vi "I2C An Out M5Stack8ChServo6DOFRobot.vi"() -> ()   [LabVIEW 2020, in "CTI-Scratchpad.lvlib"]
uses:
  CTI-Scratchpad.lvlib
  CTI/Identity.ctl
  CTI/Error Reporting.ctl
  CTI-Peripheral/Analog Output/I2C PWM/M5Stack I2C 8Ch PWM/Private/registers.ctl
  CTI-Peripheral/Analog Output/I2C PWM/M5Stack I2C 8Ch PWM/Private/GPIOOperationModes.ctl
  CTI/I2C Address.ctl
  CTI/GPIO Number.ctl
  CTI/I2C Number.ctl
  3ffc7ce8-1e09-44a0-870a-dca55598b8cb.vi
  734b1e84-ad10-4df0-a8a4-be0d7d03fa5c.vi
  755a3061-6f72-49db-9c25-f728602f264f.vi
  830ba6d0-e88d-4103-9ff4-8f2a25dc46c6.vi
  853c7eef-9088-4e40-91c4-2d7deb58307b.vi
  2fa550b4-2a40-41fb-819f-89677ffc63c5.vi
  ec3d5203-c64e-44e8-9d0a-36cdfa7c2c5f.vi
  CTI/Session/Session.lvclass
  CTI-Peripheral/Analog Output/I2C PWM/M5Stack I2C 8Ch PWM/M5Stack I2C 8Ch Servo.lvclass
  CTI/VisaComms/VisaComms.lvclass
  CTI/CTI.lvlib
panel:
  in  "Rotate to Direction 5":bool
  out "CH5Start":u8
  in  "Rotate to Direction 4":bool
  out "CH4Start":u8
  in  "Move to Direction 3":bool
  out "CH3Start":u8
  in  "Move to Direction 2":bool
  out "CH2Start":u8
  in  "Move to Direction 1":bool
  out "CH1Start":u8
  in  "Middle":bool
  out "CH0Start":u8
  in  "Rotate to Direction 0":bool
  in  "CH7":u8(slide)=90 scale=0.0..180.0
  in  "CH6":u8(slide)=90 scale=0.0..180.0
  in  "CH5":u8(knob) scale=120.0..180.0
  in  "CH4":u8(knob) scale=0.0..180.0
  in  "CH3":u8(knob)
  in  "CH2":u8(knob) scale=0.0..180.0
  in  "CH1":u8(knob) scale=0.0..180.0
  in  "CH0":u8(knob)
  out "loop":i32
  in  "stop":bool
  out "Identity":T1
  in  "Grove Connector":enum16{"I2C0", "I2C1"}(ring)
  out "error out":errorcluster
  in  "Port":refnum<visa-resource-name>="COM4"
  # "https://shop.m5stack.com/products/8-channel-servo-driver-unit-stm32f030?srsltid=AYCX9vJPlmHf0PEe2hkOf9JoORrCSCLFPOOBXTb4mmNWhcA5r_nAQ2T2"
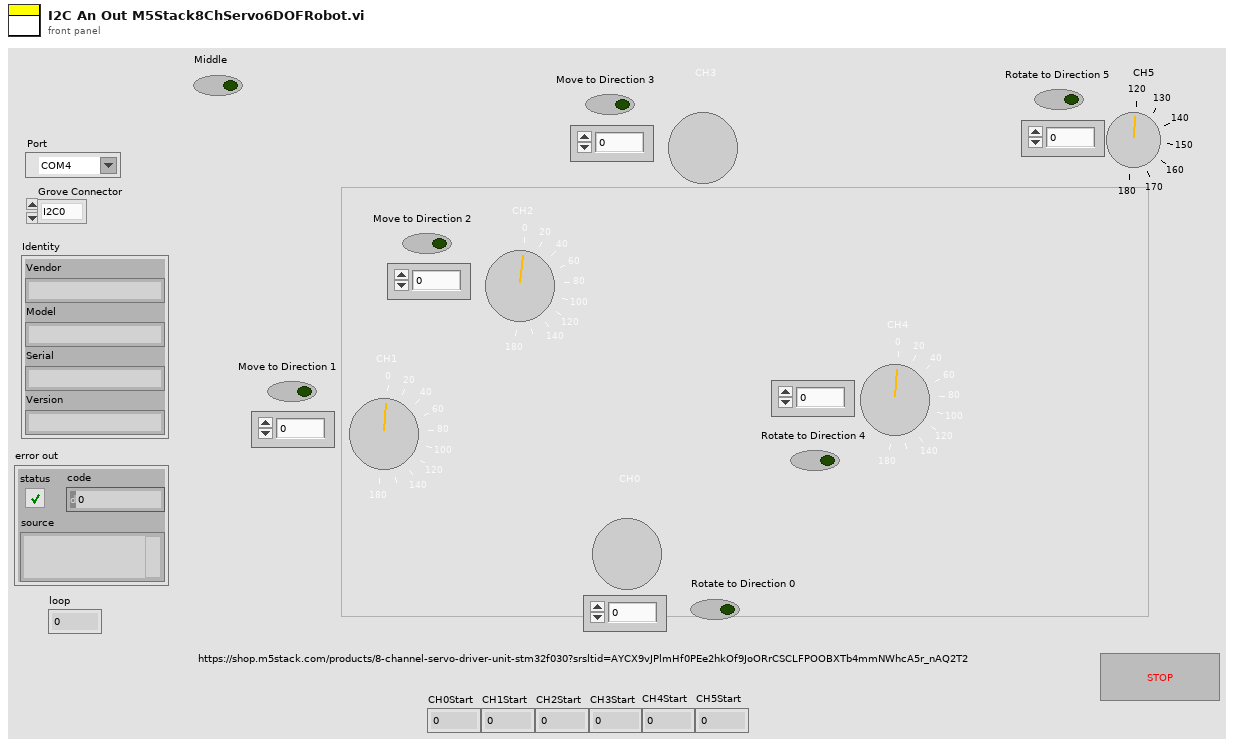
[diagram p1: front panel]
types:
  T1 = typedef "CTI.lvlib/Identity.ctl" = cluster{"Vendor":string, "Model":string, "Serial":string, "Version":string}
  T2 = typedef "CTI.lvlib/I2C Address.ctl" = u8
  T3 = typedef "CTI-Peripheral.lvlib/M5Stack I2C 8Ch Servo.lvclass/GPIOOperationModes.ctl" = u16
  T4 = typedef "CTI-Peripheral.lvlib/M5Stack I2C 8Ch Servo.lvclass/registers.ctl" = u8
  T5 = typedef "CTI.lvlib/Error Reporting.ctl" = enum16{"Minimal", "Moderate", "Full"}
  T6 = typedef "CTI.lvlib/I2C Number.ctl" = i8
  T7 = typedef "CTI.lvlib/GPIO Number.ctl" = i8
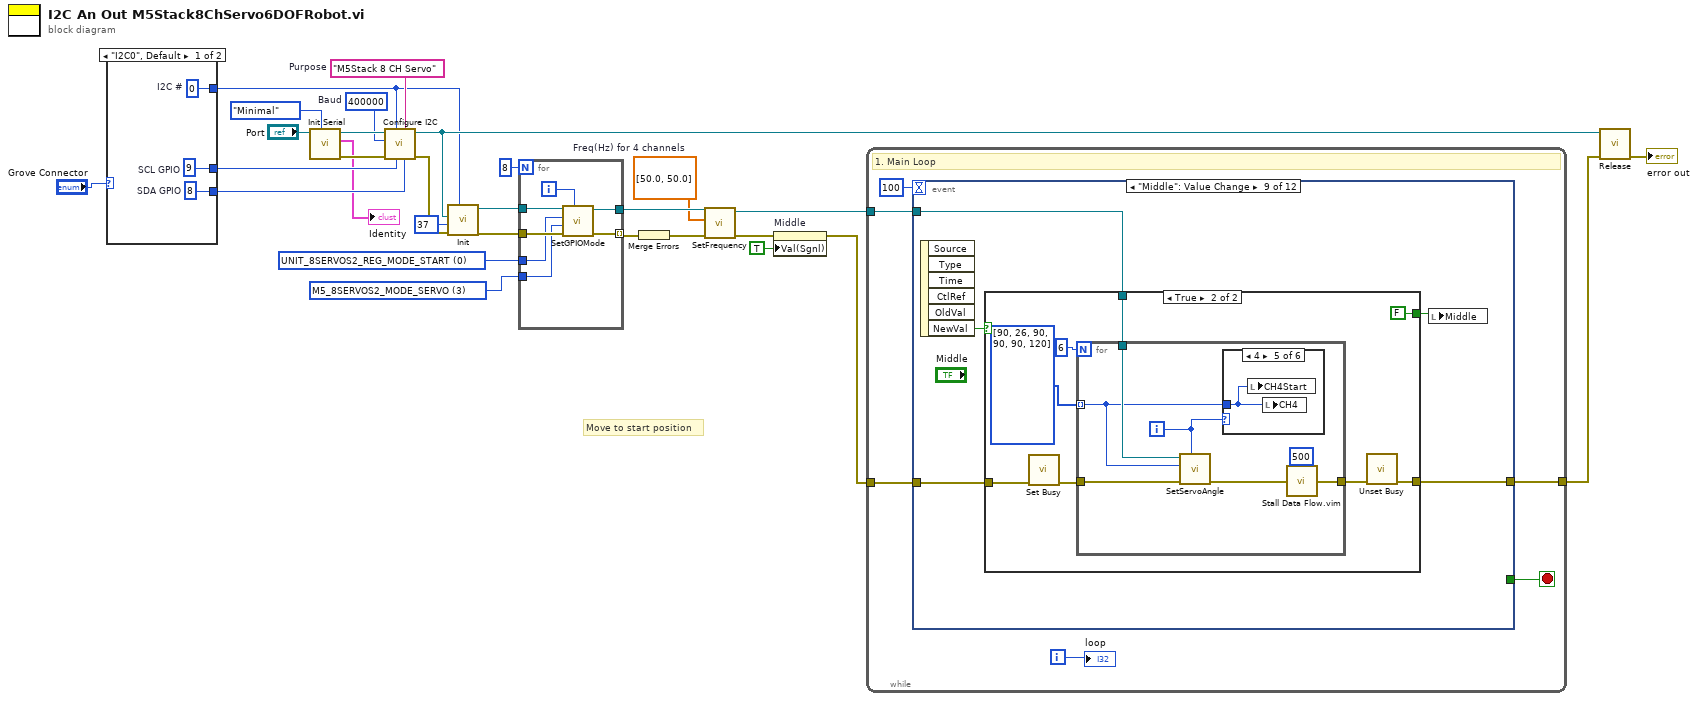
[diagram p0: block diagram]
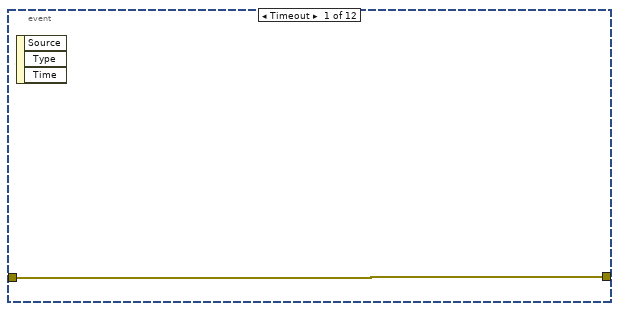
[diagram p2: hidden frame]
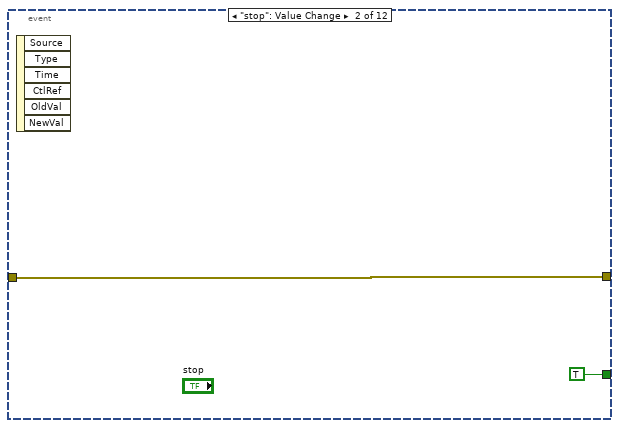
[diagram p3: hidden frame]
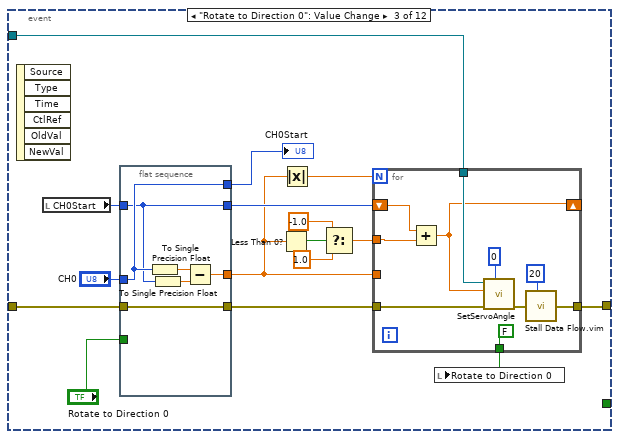
[diagram p4: hidden frame]
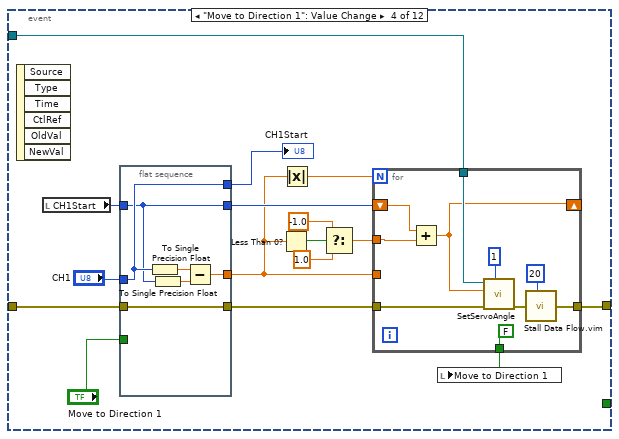
[diagram p5: hidden frame]
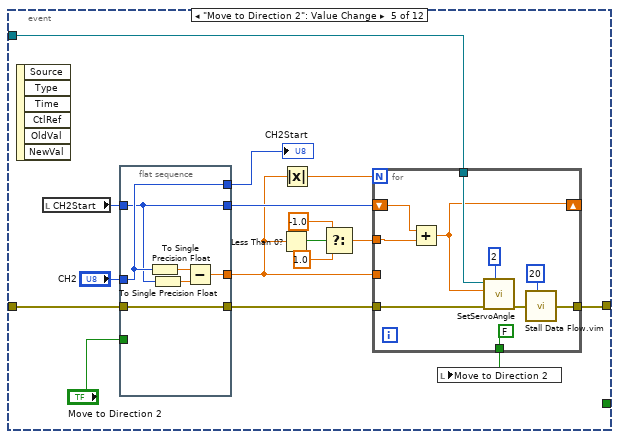
[diagram p6: hidden frame]
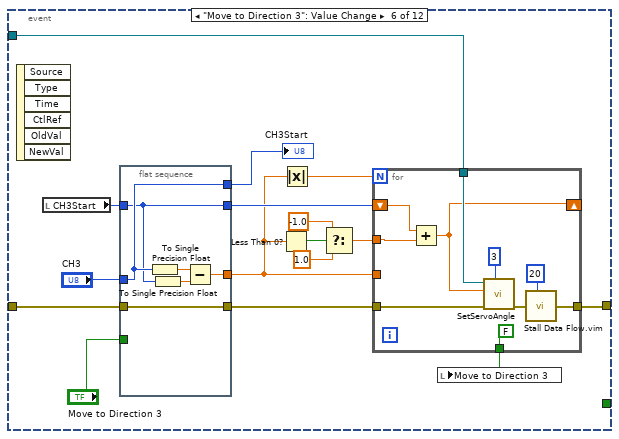
[diagram p7: hidden frame]
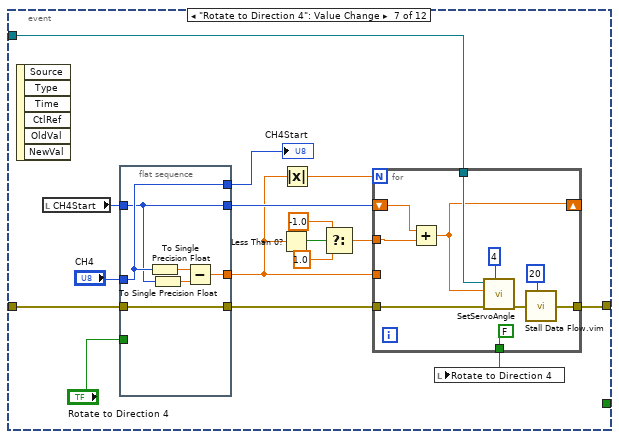
[diagram p8: hidden frame]
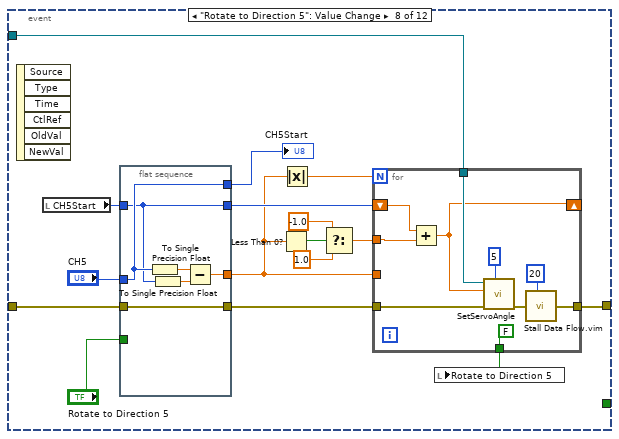
[diagram p9: hidden frame]
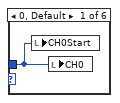
[diagram p11: hidden frame]
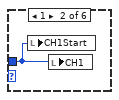
[diagram p12: hidden frame]
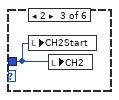
[diagram p13: hidden frame]
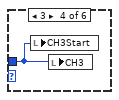
[diagram p14: hidden frame]
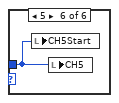
[diagram p15: hidden frame]
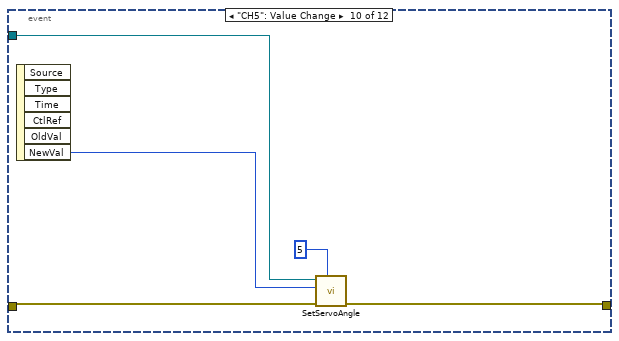
[diagram p16: hidden frame]
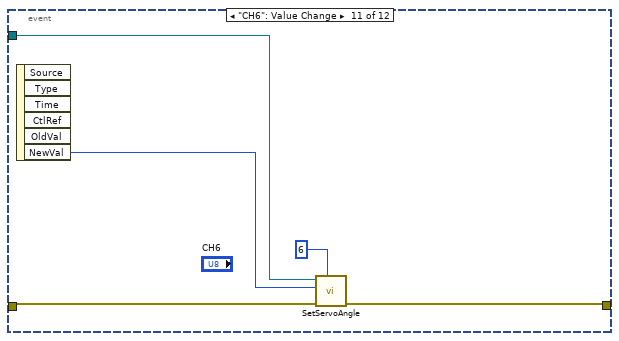
[diagram p17: hidden frame]
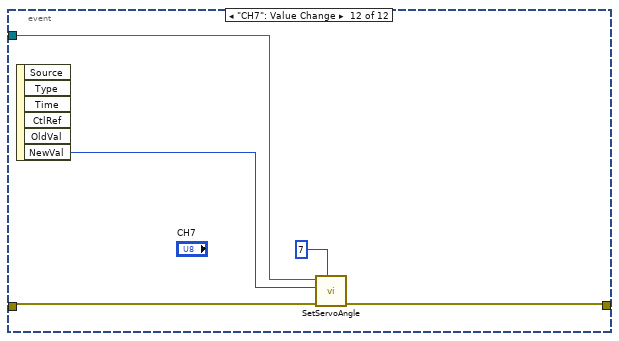
[diagram p18: hidden frame]
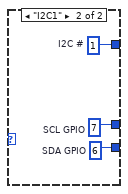
[diagram p19: hidden frame]
diagram:
  w6 = sgl[] [50.0, 50.0]  # Freq(Hz) for 4 channels
  w8 = T3 3 items=["M5_8SERVOS2_MODE_INPUT  ", "M5_8SERVOS2_MODE_OUTPUT ", "M5_8SERVOS2_MODE_ADC    ", "M5_8SERVOS2_MODE_SERVO  ", "M5_8SERVOS2_MODE_RGB    ", "M5_8SERVOS2_MODE_PWM    "] ("Op Mode")
  w9 = T4 0 items=["UNIT_8SERVOS2_REG_MODE_START"=0, "UNIT_8SERVOS2_REG_INPUT_PULL_START"=16, "UNIT_8SERVOS2_REG_INPUT_STATUS_START"=32, "UNIT_8SERVOS2_REG_OUTPUT_STATUS_START"=48, "UNIT_8SERVOS2_REG_ADC_START"=64, "UNIT_8SERVOS2_REG_SERVO_START"=80, "UNIT_8SERVOS2_REG_RGB_CONF_START"=96, "UNIT_8SERVOS2_REG_PWM_DUTY_START"=112, "UNIT_8SERVOS2_REG_RGB_BUFFER_START"=128, "UNIT_8SERVOS2_REG_TIM_FREQ_START"=208, "UNIT_8SERVOS2_REG_UID_START"=224, "UNIT_8SERVOS2_REG_UID_END"=235, "UNIT_8SERVOS2_REG_SYS_ANALOG_START"=240, "UNIT_8SERVOS2_REG_ADDR_OFFSET"=248, "UNIT_8SERVOS2_REG_I2C_ADDR_REFRESH"=252, "UNIT_8SERVOS2_REG_VERSION"=254, "UNIT_8SERVOS2_REG_I2C_ADDR"=255] ("Registers")
  w24 = "M5Stack 8 CH Servo"  # Purpose
  w25 = u32 400000  # Baud
  # "Move to start position"
  n1 = case shown="\"I2C0\", Default" "Grove Connector" {
    tunnel: [w32 w35] -> w22
    tunnel: [w31 w34] -> w21
    tunnel: [w30 w33] -> w15
    frame "I2C0", Default {
      w30 = T6 0  # I2C #
      w31 = T7 8  # SDA GPIO
      w32 = T7 9  # SCL GPIO
    }
    frame "I2C1" {
      w33 = T6 1  # I2C #
      w34 = T7 6  # SDA GPIO
      w35 = T7 7  # SCL GPIO
    }
  }
  n2 = call "Init Serial.vi"("Error Checking (Full)"=Error_Reporting."Minimal", "VISA resource name in"="Port") -> ("error out"=w26:errorcluster, "Identity"=→"Identity":T1, "Session"=w27:refnum<class "Session.lvclass">)  [unwired: 7 in]
  n3 = call "Configure I2C.vi"("SDA GPIO"=w21, "Purpose (\"I2C\")"=w24, "SCL GPIO"=w22, "I2C #"=w15, "error in (no error)"=w26, "Baud"=w25, "Session in"=w27) -> ("error out"=w16:errorcluster, "Session out"=w17:refnum<class "Session.lvclass">)  [unwired: 3 in]
  n4 = call "Init.vi"("I2C #"=w15, "error in (no error)"=w16, "Address"=T2 37, "Session In"=w17) -> ("error out"=w12:errorcluster, "M5Stack8ChPWM Out"=w14:refnum<class "M5Stack I2C 8Ch Servo.lvclass">)  [unwired: 6 in]
  n5 = for {
    N: 8 -> [_]
    tunnel: w14 -> [w42]
    tunnel: w12 -> [w40]
    tunnel: [w39] -> w11 mode=indexing
    tunnel: w9 -> [w38]
    tunnel: w8 -> [w37]
    tunnel: [w36] -> w7
    i -> [w41]
    n6 = call-dynamic "SetGPIOMode.vi"("Channel"=w41, "error in (no error)"=w40, "Op Mode"=w37, "Registers"=w38, "M5Stack I2C 8Ch Servo in"=w42) -> ("error out"=w39:errorcluster, "M5Stack I2C 8Ch Servo out"=w36:refnum<class "M5Stack I2C 8Ch Servo.lvclass">)  [unwired: 5 in]
  }
  n7 = Merge Errors(w11) -> (w10:errorcluster)
  n8 = call-dynamic "SetFrequency.vi"("error in (no error)"=w10, "Freq"=w6, "M5Stack I2C 8Ch Servo in"=w7) -> ("error out"=w3:errorcluster, "M5Stack I2C 8Ch Servo out"=w4:refnum<class "M5Stack I2C 8Ch Servo.lvclass">)  [unwired: 7 in]
  n9 = property on="Middle" class="Bool (strict)"(error in=w3, "Val(Sgnl)"=TRUE ("Value (Signaling)")) -> (error out=w2:errorcluster)  [unwired: 1 in, 1 out]
  n10 = while {
    tunnel: w2 -> [w47]
    tunnel: w4 -> [w48]
    tunnel: [w45] -> w19
    i -> [w46]
    stop <- w44 stop-if-true
    # "1. Main Loop"
    n11 = event shown="[8] \"Middle\": Value Change" {
      selector: _ -> [_ _ _ _ _ _ _ _ _ _ _ _]
      dyn-events: _ -> [_ _ _ _ _ _ _ _ _ _ _ _]
      timeout: 100 -> [_ _ _ _ _ _ _ _ _ _ _ _]
      tunnel: w48 -> [_ _ w67 w99 w131 w163 w195 w227 w247 w273 w278 w283]
      tunnel: w47 -> [w49 w50 w65 w97 w129 w161 w193 w225 w248 w275 w280 w285]
      tunnel: [w49 w50 w66 w98 w130 w162 w194 w226 w246 w274 w279 w284] -> w45
      tunnel: [_ TRUE _ _ _ _ _ _ _ _ _ _] -> w44
      event Timeout {
        n12 = event-data() -> ()  [unwired: 1 in, 3 out]
      }
      event "stop": Value Change {
        n13 = event-data() -> ()  [unwired: 1 in, 6 out]
      }
      event "Rotate to Direction 0": Value Change {
        n14 = event-data() -> ()  [unwired: 1 in, 6 out]
        n15 = local read "CH0Start"() -> (w63:u8)
        n16 = flat-sequence {
          tunnel: w65 -> [w73]
          tunnel: "CH0" -> [w72]
          tunnel: w63 -> [w71]
          tunnel: [w73] -> w62
          tunnel: [w72] -> w61
          tunnel: [w71] -> w60
          tunnel: [w70] -> w58
          tunnel: "Rotate to Direction 0" -> [_]
          frame #0 {
            n17 = To Single Precision Float(number=w72) -> (single precision float=w68:sgl)
            n18 = To Single Precision Float(number=w71) -> (single precision float=w69:sgl)
            n19 = Subtract(x=w68, y=w69) -> (x-y=w70:sgl)
          }
        }
        n20 = Less Than 0?(x=w58) -> (x < 0?=w57:bool)
        n21 = Absolute Value(x=w58) -> (abs(x)=w59:sgl)
        n22 = Select(t=-1.0, s=w57, f=1.0) -> (s? t:f=w54:dbl)
        n23 = for {
          N: w59 -> [_]
          tunnel: w67 -> [w82]
          tunnel: w62 -> [w83]
          tunnel: [w79] -> w66
          tunnel: w58 -> [_]
          shift-right: [w75] -> _
          shift-left: w60 -> [w76]
          tunnel: w54 -> [w77]
          tunnel: [FALSE] -> w52
          n24 = Add(x=w76, y=w77) -> (x+y=w75:dbl)
          n25 = call-dynamic "SetServoAngle.vi"("Channel"=u8 0, "error in (no error)"=w83, "Angle"=w75, "M5Stack I2C 8Ch Servo in"=w82) -> ("error out"=w80:errorcluster)  [unwired: 6 in, 1 out]
          n26 = call "Stall Data Flow.vim"("value in"=w80, "milliseconds to wait"=u32 20) -> ("value out"=w79:errorcluster)  [unwired: 1 out]
        }
        n27 = local write "Rotate to Direction 0"(w52) -> ()
        "CH0Start" <- w61
      }
      event "Move to Direction 1": Value Change {
        n28 = event-data() -> ()  [unwired: 1 in, 6 out]
        n29 = local read "CH1Start"() -> (w96:u8)
        n30 = flat-sequence {
          tunnel: w97 -> [w105]
          tunnel: "CH1" -> [w104]
          tunnel: w96 -> [w103]
          tunnel: [w105] -> w95
          tunnel: [w104] -> w94
          tunnel: [w103] -> w93
          tunnel: [w102] -> w91
          tunnel: "Move to Direction 1" -> [_]
          frame #0 {
            n31 = To Single Precision Float(number=w104) -> (single precision float=w100:sgl)
            n32 = To Single Precision Float(number=w103) -> (single precision float=w101:sgl)
            n33 = Subtract(x=w100, y=w101) -> (x-y=w102:sgl)
          }
        }
        n34 = Less Than 0?(x=w91) -> (x < 0?=w90:bool)
        n35 = Absolute Value(x=w91) -> (abs(x)=w92:sgl)
        n36 = Select(t=-1.0, s=w90, f=1.0) -> (s? t:f=w87:dbl)
        n37 = for {
          N: w92 -> [_]
          tunnel: w99 -> [w114]
          tunnel: w95 -> [w115]
          tunnel: [w111] -> w98
          tunnel: w91 -> [_]
          shift-right: [w107] -> _
          shift-left: w93 -> [w108]
          tunnel: w87 -> [w109]
          tunnel: [FALSE] -> w85
          n38 = Add(x=w108, y=w109) -> (x+y=w107:dbl)
          n39 = call-dynamic "SetServoAngle.vi"("Channel"=u8 1, "error in (no error)"=w115, "Angle"=w107, "M5Stack I2C 8Ch Servo in"=w114) -> ("error out"=w112:errorcluster)  [unwired: 6 in, 1 out]
          n40 = call "Stall Data Flow.vim"("value in"=w112, "milliseconds to wait"=u32 20) -> ("value out"=w111:errorcluster)  [unwired: 1 out]
        }
        n41 = local write "Move to Direction 1"(w85) -> ()
        "CH1Start" <- w94
      }
      event "Move to Direction 2": Value Change {
        n42 = event-data() -> ()  [unwired: 1 in, 6 out]
        n43 = local read "CH2Start"() -> (w128:u8)
        n44 = flat-sequence {
          tunnel: w129 -> [w137]
          tunnel: "CH2" -> [w136]
          tunnel: w128 -> [w135]
          tunnel: [w137] -> w127
          tunnel: [w136] -> w126
          tunnel: [w135] -> w125
          tunnel: [w134] -> w123
          tunnel: "Move to Direction 2" -> [_]
          frame #0 {
            n45 = To Single Precision Float(number=w136) -> (single precision float=w132:sgl)
            n46 = To Single Precision Float(number=w135) -> (single precision float=w133:sgl)
            n47 = Subtract(x=w132, y=w133) -> (x-y=w134:sgl)
          }
        }
        n48 = Less Than 0?(x=w123) -> (x < 0?=w122:bool)
        n49 = Absolute Value(x=w123) -> (abs(x)=w124:sgl)
        n50 = Select(t=-1.0, s=w122, f=1.0) -> (s? t:f=w119:dbl)
        n51 = for {
          N: w124 -> [_]
          tunnel: w131 -> [w146]
          tunnel: w127 -> [w147]
          tunnel: [w143] -> w130
          tunnel: w123 -> [_]
          shift-right: [w139] -> _
          shift-left: w125 -> [w140]
          tunnel: w119 -> [w141]
          tunnel: [FALSE] -> w117
          n52 = Add(x=w140, y=w141) -> (x+y=w139:dbl)
          n53 = call-dynamic "SetServoAngle.vi"("Channel"=u8 2, "error in (no error)"=w147, "Angle"=w139, "M5Stack I2C 8Ch Servo in"=w146) -> ("error out"=w144:errorcluster)  [unwired: 6 in, 1 out]
          n54 = call "Stall Data Flow.vim"("value in"=w144, "milliseconds to wait"=u32 20) -> ("value out"=w143:errorcluster)  [unwired: 1 out]
        }
        n55 = local write "Move to Direction 2"(w117) -> ()
        "CH2Start" <- w126
      }
      event "Move to Direction 3": Value Change {
        n56 = event-data() -> ()  [unwired: 1 in, 6 out]
        n57 = local read "CH3Start"() -> (w160:u8)
        n58 = flat-sequence {
          tunnel: w161 -> [w169]
          tunnel: "CH3" -> [w168]
          tunnel: w160 -> [w167]
          tunnel: [w169] -> w159
          tunnel: [w168] -> w158
          tunnel: [w167] -> w157
          tunnel: [w166] -> w155
          tunnel: "Move to Direction 3" -> [_]
          frame #0 {
            n59 = To Single Precision Float(number=w168) -> (single precision float=w164:sgl)
            n60 = To Single Precision Float(number=w167) -> (single precision float=w165:sgl)
            n61 = Subtract(x=w164, y=w165) -> (x-y=w166:sgl)
          }
        }
        n62 = Less Than 0?(x=w155) -> (x < 0?=w154:bool)
        n63 = Absolute Value(x=w155) -> (abs(x)=w156:sgl)
        n64 = Select(t=-1.0, s=w154, f=1.0) -> (s? t:f=w151:dbl)
        n65 = for {
          N: w156 -> [_]
          tunnel: w163 -> [w178]
          tunnel: w159 -> [w179]
          tunnel: [w175] -> w162
          tunnel: w155 -> [_]
          shift-right: [w171] -> _
          shift-left: w157 -> [w172]
          tunnel: w151 -> [w173]
          tunnel: [FALSE] -> w149
          n66 = Add(x=w172, y=w173) -> (x+y=w171:dbl)
          n67 = call-dynamic "SetServoAngle.vi"("Channel"=u8 3, "error in (no error)"=w179, "Angle"=w171, "M5Stack I2C 8Ch Servo in"=w178) -> ("error out"=w176:errorcluster)  [unwired: 6 in, 1 out]
          n68 = call "Stall Data Flow.vim"("value in"=w176, "milliseconds to wait"=u32 20) -> ("value out"=w175:errorcluster)  [unwired: 1 out]
        }
        n69 = local write "Move to Direction 3"(w149) -> ()
        "CH3Start" <- w158
      }
      event "Rotate to Direction 4": Value Change {
        n70 = event-data() -> ()  [unwired: 1 in, 6 out]
        n71 = local read "CH4Start"() -> (w192:u8)
        n72 = flat-sequence {
          tunnel: w193 -> [w201]
          tunnel: "CH4" -> [w200]
          tunnel: w192 -> [w199]
          tunnel: [w201] -> w191
          tunnel: [w200] -> w190
          tunnel: [w199] -> w189
          tunnel: [w198] -> w187
          tunnel: "Rotate to Direction 4" -> [_]
          frame #0 {
            n73 = To Single Precision Float(number=w200) -> (single precision float=w196:sgl)
            n74 = To Single Precision Float(number=w199) -> (single precision float=w197:sgl)
            n75 = Subtract(x=w196, y=w197) -> (x-y=w198:sgl)
          }
        }
        n76 = Less Than 0?(x=w187) -> (x < 0?=w186:bool)
        n77 = Absolute Value(x=w187) -> (abs(x)=w188:sgl)
        n78 = Select(t=-1.0, s=w186, f=1.0) -> (s? t:f=w183:dbl)
        n79 = for {
          N: w188 -> [_]
          tunnel: w195 -> [w210]
          tunnel: w191 -> [w211]
          tunnel: [w207] -> w194
          tunnel: w187 -> [_]
          shift-right: [w203] -> _
          shift-left: w189 -> [w204]
          tunnel: w183 -> [w205]
          tunnel: [FALSE] -> w181
          n80 = Add(x=w204, y=w205) -> (x+y=w203:dbl)
          n81 = call-dynamic "SetServoAngle.vi"("Channel"=u8 4, "error in (no error)"=w211, "Angle"=w203, "M5Stack I2C 8Ch Servo in"=w210) -> ("error out"=w208:errorcluster)  [unwired: 6 in, 1 out]
          n82 = call "Stall Data Flow.vim"("value in"=w208, "milliseconds to wait"=u32 20) -> ("value out"=w207:errorcluster)  [unwired: 1 out]
        }
        n83 = local write "Rotate to Direction 4"(w181) -> ()
        "CH4Start" <- w190
      }
      event "Rotate to Direction 5": Value Change {
        n84 = event-data() -> ()  [unwired: 1 in, 6 out]
        n85 = local read "CH5Start"() -> (w224:u8)
        n86 = flat-sequence {
          tunnel: w225 -> [w233]
          tunnel: "CH5" -> [w232]
          tunnel: w224 -> [w231]
          tunnel: [w233] -> w223
          tunnel: [w232] -> w222
          tunnel: [w231] -> w221
          tunnel: [w230] -> w219
          tunnel: "Rotate to Direction 5" -> [_]
          frame #0 {
            n87 = To Single Precision Float(number=w232) -> (single precision float=w228:sgl)
            n88 = To Single Precision Float(number=w231) -> (single precision float=w229:sgl)
            n89 = Subtract(x=w228, y=w229) -> (x-y=w230:sgl)
          }
        }
        n90 = Less Than 0?(x=w219) -> (x < 0?=w218:bool)
        n91 = Absolute Value(x=w219) -> (abs(x)=w220:sgl)
        n92 = Select(t=-1.0, s=w218, f=1.0) -> (s? t:f=w215:dbl)
        n93 = for {
          N: w220 -> [_]
          tunnel: w227 -> [w242]
          tunnel: w223 -> [w243]
          tunnel: [w239] -> w226
          tunnel: w219 -> [_]
          shift-right: [w235] -> _
          shift-left: w221 -> [w236]
          tunnel: w215 -> [w237]
          tunnel: [FALSE] -> w213
          n94 = Add(x=w236, y=w237) -> (x+y=w235:dbl)
          n95 = call-dynamic "SetServoAngle.vi"("Channel"=u8 5, "error in (no error)"=w243, "Angle"=w235, "M5Stack I2C 8Ch Servo in"=w242) -> ("error out"=w240:errorcluster)  [unwired: 6 in, 1 out]
          n96 = call "Stall Data Flow.vim"("value in"=w240, "milliseconds to wait"=u32 20) -> ("value out"=w239:errorcluster)  [unwired: 1 out]
        }
        n97 = local write "Rotate to Direction 5"(w213) -> ()
        "CH5Start" <- w222
      }
      event "Middle": Value Change {
        n98 = event-data() -> ("NewVal"=w245:bool)  [unwired: 1 in, 5 out]
        n99 = case shown="True" w245 {
          tunnel: w248 -> [w249 w257]
          tunnel: w247 -> [_ w255]
          tunnel: [w249 w252] -> w246
          tunnel: [_ FALSE] -> w244
          frame False {
          }
          frame True {
            n100 = call <vilib>:"Set Busy.vi"("error in (no error)"=w257) -> ("error out"=w253:errorcluster)  [unwired: 9 in, 1 out]
            n101 = for {
              N: 6 -> [_]
              tunnel: w255 -> [w262]
              tunnel: w253 -> [w264]
              tunnel: [w261] -> w256
              tunnel: u8[] [90, 26, 90, 90, 90, 120] -> [w258] mode=indexing
              i -> [w259]
              n102 = call-dynamic "SetServoAngle.vi"("Channel"=w259, "error in (no error)"=w264, "Angle"=w258, "M5Stack I2C 8Ch Servo in"=w262) -> ("error out"=w263:errorcluster)  [unwired: 6 in, 1 out]
              n103 = case shown="4" w259 {
                tunnel: w258 -> [w265 w266 w267 w268 w269 w270]
                frame 0, Default {
                  n104 = local write "CH0Start"(w265) -> ()
                  n105 = local write "CH0"(w265) -> ()
                }
                frame 1 {
                  n106 = local write "CH1Start"(w266) -> ()
                  n107 = local write "CH1"(w266) -> ()
                }
                frame 2 {
                  n108 = local write "CH2Start"(w267) -> ()
                  n109 = local write "CH2"(w267) -> ()
                }
                frame 3 {
                  n110 = local write "CH3Start"(w268) -> ()
                  n111 = local write "CH3"(w268) -> ()
                }
                frame 4 {
                  n112 = local write "CH4Start"(w269) -> ()
                  n113 = local write "CH4"(w269) -> ()
                }
                frame 5 {
                  n114 = local write "CH5Start"(w270) -> ()
                  n115 = local write "CH5"(w270) -> ()
                }
              }
              n116 = call "Stall Data Flow.vim"("value in"=w263, "milliseconds to wait"=u32 500) -> ("value out"=w261:errorcluster)  [unwired: 1 out]
            }
            n117 = call <vilib>:"Unset Busy.vi"("error in (no error)"=w256) -> ("error out"=w252:errorcluster)  [unwired: 10 in]
          }
        }
        n118 = local write "Middle"(w244) -> ()
      }
      event "CH5": Value Change {
        n119 = event-data() -> ("NewVal"=w272:u8)  [unwired: 1 in, 5 out]
        n120 = call-dynamic "SetServoAngle.vi"("Channel"=u8 5, "error in (no error)"=w275, "Angle"=w272, "M5Stack I2C 8Ch Servo in"=w273) -> ("error out"=w274:errorcluster)  [unwired: 6 in, 1 out]
      }
      event "CH6": Value Change {
        n121 = event-data() -> ("NewVal"=w277:u8)  [unwired: 1 in, 5 out]
        n122 = call-dynamic "SetServoAngle.vi"("Channel"=u8 6, "error in (no error)"=w280, "Angle"=w277, "M5Stack I2C 8Ch Servo in"=w278) -> ("error out"=w279:errorcluster)  [unwired: 6 in, 1 out]
      }
      event "CH7": Value Change {
        n123 = event-data() -> ("NewVal"=w282:u8)  [unwired: 1 in, 5 out]
        n124 = call-dynamic "SetServoAngle.vi"("Channel"=u8 7, "error in (no error)"=w285, "Angle"=w282, "M5Stack I2C 8Ch Servo in"=w283) -> ("error out"=w284:errorcluster)  [unwired: 6 in, 1 out]
      }
    }
    "loop" <- w46
  }
  n125 = call-dynamic "Release.vi"("error in (no error)"=w19, "Session in"=w17) -> ("error out"=→"error out":errorcluster)  [unwired: 9 in]
